vi "set OBW - RBW or VBW.vi"(6 "BW Auto?":bool, 8 "error in (no error)":errorcluster, 9 "BW Type":T1, 10 "BW Value (Hz)":dbl format="%#_6p", 11 "Keysight 9020A in":refnum<class "Keysight 9020A.lvclass">) -> (0 "error out":errorcluster, 3 "Keysight 9020A out":refnum<class "Keysight 9020A.lvclass">)   [LabVIEW 2023, in "Spectrum Analyzer.lvlib" / "Keysight 9020A.lvclass"]
uses:
  Keysight 9020A.lvclass
  Keysight 9020A.lvclass/Keysight 9020A.ctl
  TYPE DEFINITION/TYPE RBW and VBW Select.ctl
  Spectrum Analyzer.lvlib
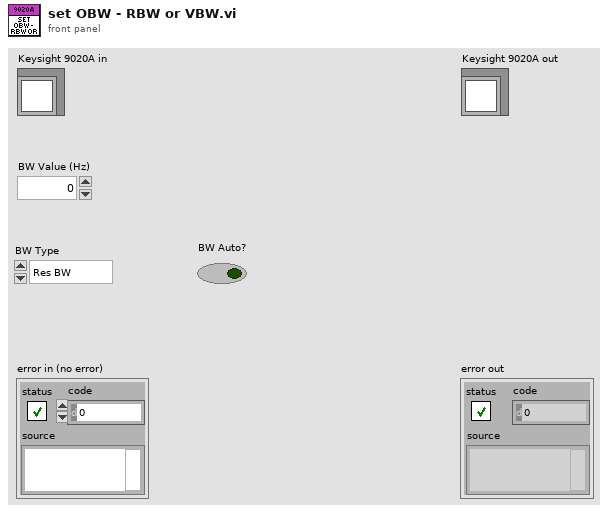
[diagram p1: front panel]
types:
  T1 = typedef "Spectrum Analyzer.lvlib/TYPE RBW and VBW Select.ctl" = enum16{"Res BW", "Video BW"}
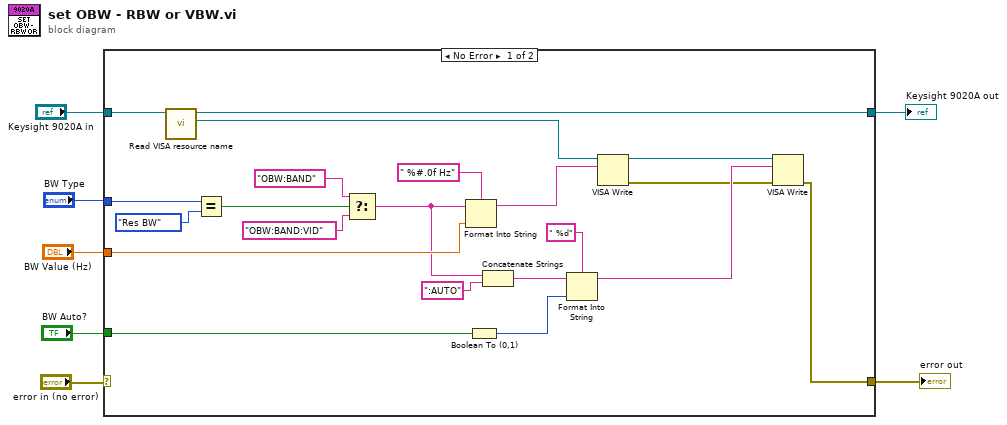
[diagram p0: block diagram]
diagram:
  n1 = case shown="No Error" "error in (no error)" {
    selector: "error in (no error)" -> [_ w29]
    tunnel: "Keysight 9020A in" -> [w28 w30]
    tunnel: [w27 w30] -> w6
    tunnel: [w19 w29] -> w4
    tunnel: "BW Auto?" -> [w9 _]
    tunnel: "BW Value (Hz)" -> [w13 _]
    tunnel: "BW Type" -> [w18 _]
    frame No Error {
      n2 = call "Read VISA resource name.vi"("Keysight 9020A in"=w28) -> ("VISA resource name"=w26:refnum<visa-resource-name>, "Keysight 9020A out"=w27:refnum<class "Keysight 9020A.lvclass">)  [unwired: 8 in, 1 out]
      n3 = Equal?(x=w18, y=TYPE_RBW_and_VBW_Select."Res BW") -> (x = y?=w16:bool)
      n4 = Select(t="OBW:BAND", s=w16, f="OBW:BAND:VID") -> (s? t:f=w12:string)
      n5 = Format Into String(format string=" %#.0f Hz", initial string=w12, w13) -> (resulting string=w25:string)  [unwired: 1 in, 1 out]
      n6 = Boolean To (0,1)(Boolean=w9) -> (0, 1=w8:i16)
      n7 = Concatenate Strings(w12, ":AUTO" ("string")) -> (w10:string)
      n8 = Format Into String(format string=" %d", initial string=w10, w8) -> (resulting string=w22:string)  [unwired: 1 in, 1 out]
      n9 = VISA Write(VISA resource name=w26, write buffer=w25) -> (VISA resource name out=w21:refnum<visa-resource-name>, error out=w20:errorcluster)  [unwired: 1 in, 1 out]
      n10 = VISA Write(VISA resource name=w21, write buffer=w22, error in (no error)=w20) -> (error out=w19:errorcluster)  [unwired: 2 out]
    }
    frame Error {
    }
  }
  "error out" <- w4
  "Keysight 9020A out" <- w6
